vi "UI_Settings_Layout.vi"(11 "error in":errorcluster) -> (4 "Specs":T1(array[cluster]), 15 "error out":errorcluster)   [LabVIEW 2026]
doc: "설정 화면 버튼/글자 배치표. Group 0=모드, 1=선공, 2=난이도, 3=규칙, 4=게임 시작."
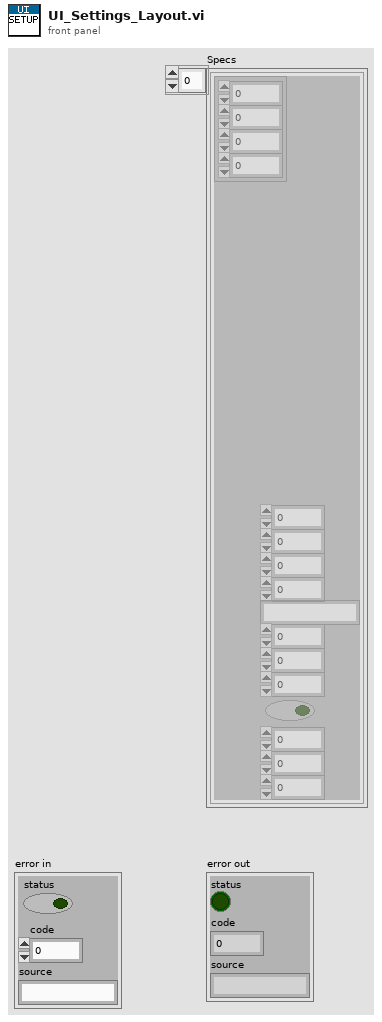
[diagram p1: front panel]
types:
  T1 = cluster{"Rect":cluster{"left":i16, "top":i16, "right":i16, "bottom":i16}, "Fill":u32, "Fill Sel":u32, "Border":u32, "Border Sel":u32, "Text":string, "Text Color":u32, "Text Sel":u32, "Size":i16, "Bold":bool, "Group":i32, "Value":i32, "Radius":i16}[]
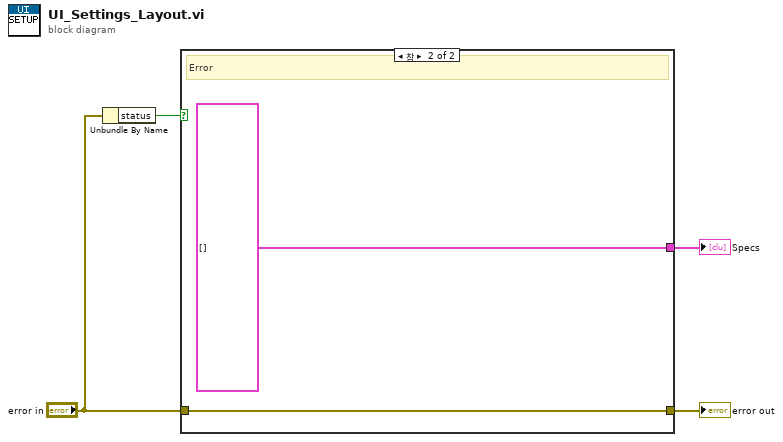
[diagram p0: block diagram]
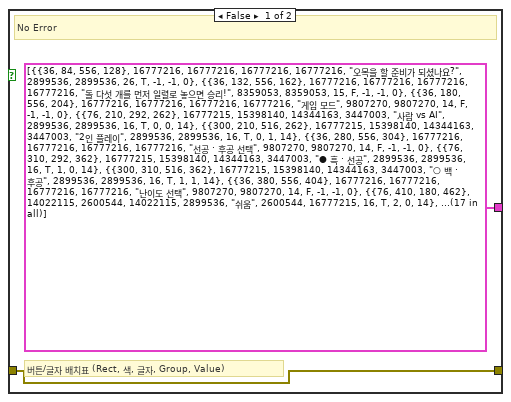
[diagram p2: hidden frame]
diagram:
  n1 = Unbundle By Name("error in") -> ("status"=w2:bool)
  n2 = case shown="참" w2 {
    tunnel: "error in" -> [w5 w7]
    tunnel: [T1 [{"Rect"={"left"=36, "top"=84, "right"=556, "bottom"=128}, "Fill"=16777216, "Fill Sel"=16777216, "Border"=16777216, "Border Sel"=16777216, "Text"="오목을 할 준비가 되셨나요?", "Text Color"=2899536, "Text Sel"=2899536, "Size"=26, "Bold"=TRUE, "Group"=-1, "Value"=-1, "Radius"=0}, {"Rect"={"left"=36, "top"=132, "right"=556, "bottom"=162}, "Fill"=16777216, "Fill Sel"=16777216, "Border"=16777216, "Border Sel"=16777216, "Text"="돌 다섯 개를 먼저 일렬로 놓으면 승리!", "Text Color"=8359053, "Text Sel"=8359053, "Size"=15, "Bold"=FALSE, "Group"=-1, "Value"=-1, "Radius"=0}, {"Rect"={"left"=36, "top"=180, "right"=556, "bottom"=204}, "Fill"=16777216, "Fill Sel"=16777216, "Border"=16777216, "Border Sel"=16777216, "Text"="게임 모드", "Text Color"=9807270, "Text Sel"=9807270, "Size"=14, "Bold"=FALSE, "Group"=-1, "Value"=-1, "Radius"=0}, {"Rect"={"left"=76, "top"=210, "right"=292, "bottom"=262}, "Fill"=16777215, "Fill Sel"=15398140, "Border"=14344163, "Border Sel"=3447003, "Text"="사람 vs AI", "Text Color"=2899536, "Text Sel"=2899536, "Size"=16, "Bold"=TRUE, "Group"=0, "Value"=0, "Radius"=14}, {"Rect"={"left"=300, "top"=210, "right"=516, "bottom"=262}, "Fill"=16777215, "Fill Sel"=15398140, "Border"=14344163, "Border Sel"=3447003, "Text"="2인 플레이", "Text Color"=2899536, "Text Sel"=2899536, "Size"=16, "Bold"=TRUE, "Group"=0, "Value"=1, "Radius"=14}, {"Rect"={"left"=36, "top"=280, "right"=556, "bottom"=304}, "Fill"=16777216, "Fill Sel"=16777216, "Border"=16777216, "Border Sel"=16777216, "Text"="선공 · 후공 선택", "Text Color"=9807270, "Text Sel"=9807270, "Size"=14, "Bold"=FALSE, "Group"=-1, "Value"=-1, "Radius"=0}, {"Rect"={"left"=76, "top"=310, "right"=292, "bottom"=362}, "Fill"=16777215, "Fill Sel"=15398140, "Border"=14344163, "Border Sel"=3447003, "Text"="● 흑 · 선공", "Text Color"=2899536, "Text Sel"=2899536, "Size"=16, "Bold"=TRUE, "Group"=1, "Value"=0, "Radius"=14}, {"Rect"={"left"=300, "top"=310, "right"=516, "bottom"=362}, "Fill"=16777215, "Fill Sel"=15398140, "Border"=14344163, "Border Sel"=3447003, "Text"="○ 백 · 후공", "Text Color"=2899536, "Text Sel"=2899536, "Size"=16, "Bold"=TRUE, "Group"=1, "Value"=1, "Radius"=14}, {"Rect"={"left"=36, "top"=380, "right"=556, "bottom"=404}, "Fill"=16777216, "Fill Sel"=16777216, "Border"=16777216, "Border Sel"=16777216, "Text"="난이도 선택", "Text Color"=9807270, "Text Sel"=9807270, "Size"=14, "Bold"=FALSE, "Group"=-1, "Value"=-1, "Radius"=0}, {"Rect"={"left"=76, "top"=410, "right"=180, "bottom"=462}, "Fill"=14022115, "Fill Sel"=2600544, "Border"=14022115, "Border Sel"=2899536, "Text"="쉬움", "Text Color"=2600544, "Text Sel"=16777215, "Size"=16, "Bold"=TRUE, "Group"=2, "Value"=0, "Radius"=14}, {"Rect"={"left"=188, "top"=410, "right"=292, "bottom"=462}, "Fill"=14084856, "Fill Sel"=3447003, "Border"=14084856, "Border Sel"=2899536, "Text"="보통", "Text Color"=3447003, "Text Sel"=16777215, "Size"=16, "Bold"=TRUE, "Group"=2, "Value"=1, "Radius"=14}, {"Rect"={"left"=300, "top"=410, "right"=404, "bottom"=462}, "Fill"=16442835, "Fill Sel"=15105570, "Border"=16442835, "Border Sel"=2899536, "Text"="어려움", "Text Color"=15105570, "Text Sel"=16777215, "Size"=16, "Bold"=TRUE, "Group"=2, "Value"=2, "Radius"=14}, {"Rect"={"left"=412, "top"=410, "right"=516, "bottom"=462}, "Fill"=16440280, "Fill Sel"=15158332, "Border"=16440280, "Border Sel"=2899536, "Text"="마스터", "Text Color"=15158332, "Text Sel"=16777215, "Size"=16, "Bold"=TRUE, "Group"=2, "Value"=3, "Radius"=14}, {"Rect"={"left"=36, "top"=480, "right"=556, "bottom"=504}, "Fill"=16777216, "Fill Sel"=16777216, "Border"=16777216, "Border Sel"=16777216, "Text"="규칙", "Text Color"=9807270, "Text Sel"=9807270, "Size"=14, "Bold"=FALSE, "Group"=-1, "Value"=-1, "Radius"=0}, {"Rect"={"left"=76, "top"=510, "right"=292, "bottom"=562}, "Fill"=16777215, "Fill Sel"=15398140, "Border"=14344163, "Border Sel"=3447003, "Text"="렌주룰 (흑 금수)", "Text Color"=2899536, "Text Sel"=2899536, "Size"=16, "Bold"=TRUE, "Group"=3, "Value"=1, "Radius"=14}, {"Rect"={"left"=300, "top"=510, "right"=516, "bottom"=562}, "Fill"=16777215, "Fill Sel"=15398140, "Border"=14344163, "Border Sel"=3447003, "Text"="자유룰 (제한 없음)", "Text Color"=2899536, "Text Sel"=2899536, "Size"=16, "Bold"=TRUE, "Group"=3, "Value"=0, "Radius"=14}, {"Rect"={"left"=76, "top"=600, "right"=516, "bottom"=670}, "Fill"=2899536, "Fill Sel"=2899536, "Border"=2899536, "Border Sel"=2899536, "Text"="게임 시작", "Text Color"=16777215, "Text Sel"=16777215, "Size"=22, "Bold"=TRUE, "Group"=4, "Value"=-1, "Radius"=14}] ("Layout") T1 []] -> w3
    tunnel: [w5 w7] -> w4
    frame False {
      # "버튼/글자 배치표 (Rect, 색, 글자, Group, Value)"
      # "No Error"
    }
    frame True {
      # "Error"
    }
  }
  "Specs" <- w3
  "error out" <- w4
